vi "PicoReadPicoStreamingBuffers.vi"(1 "enabled array":i16[](array[numeric]), 2 "Buffer and Transfer Settings":T2 {"Down-Sample Mode" items=["None", "Aggregate", "Decimate", "Average"]; "Down Sample Ratio" step=1; "Samples" format="%_6p"}, 3 "Variant":string, 5 "Pointer array":u64[][](array[numeric]), 7 "Offset Index":u32, 9 "Number of Samples":u32, 11 "error in (no error)":errorcluster) -> (6 "Buffers (Max or non-aggregated)":T1, 8 "Buffers (Min)":T1, 15 "error out":errorcluster)   [LabVIEW 2009]
doc: "Read data from Picodata buffers for streaming examples"
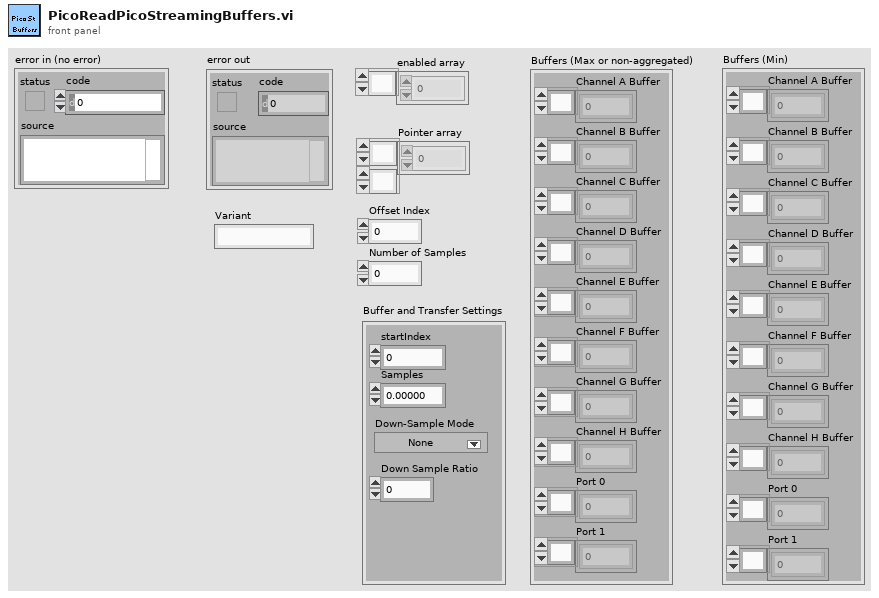
[diagram p1: front panel]
types:
  T1 = cluster{"Channel A Buffer":i16[], "Channel B Buffer":i16[], "Channel C Buffer":i16[], "Channel D Buffer":i16[], "Channel E Buffer":i16[], "Channel F Buffer":i16[], "Channel G Buffer":i16[], "Channel H Buffer":i16[], "Port 0":i16[], "Port 1":i16[]}
  T2 = cluster{"startIndex":u64, "Samples":u64, "Down Sample Ratio":u64, "Down-Sample Mode":u32}
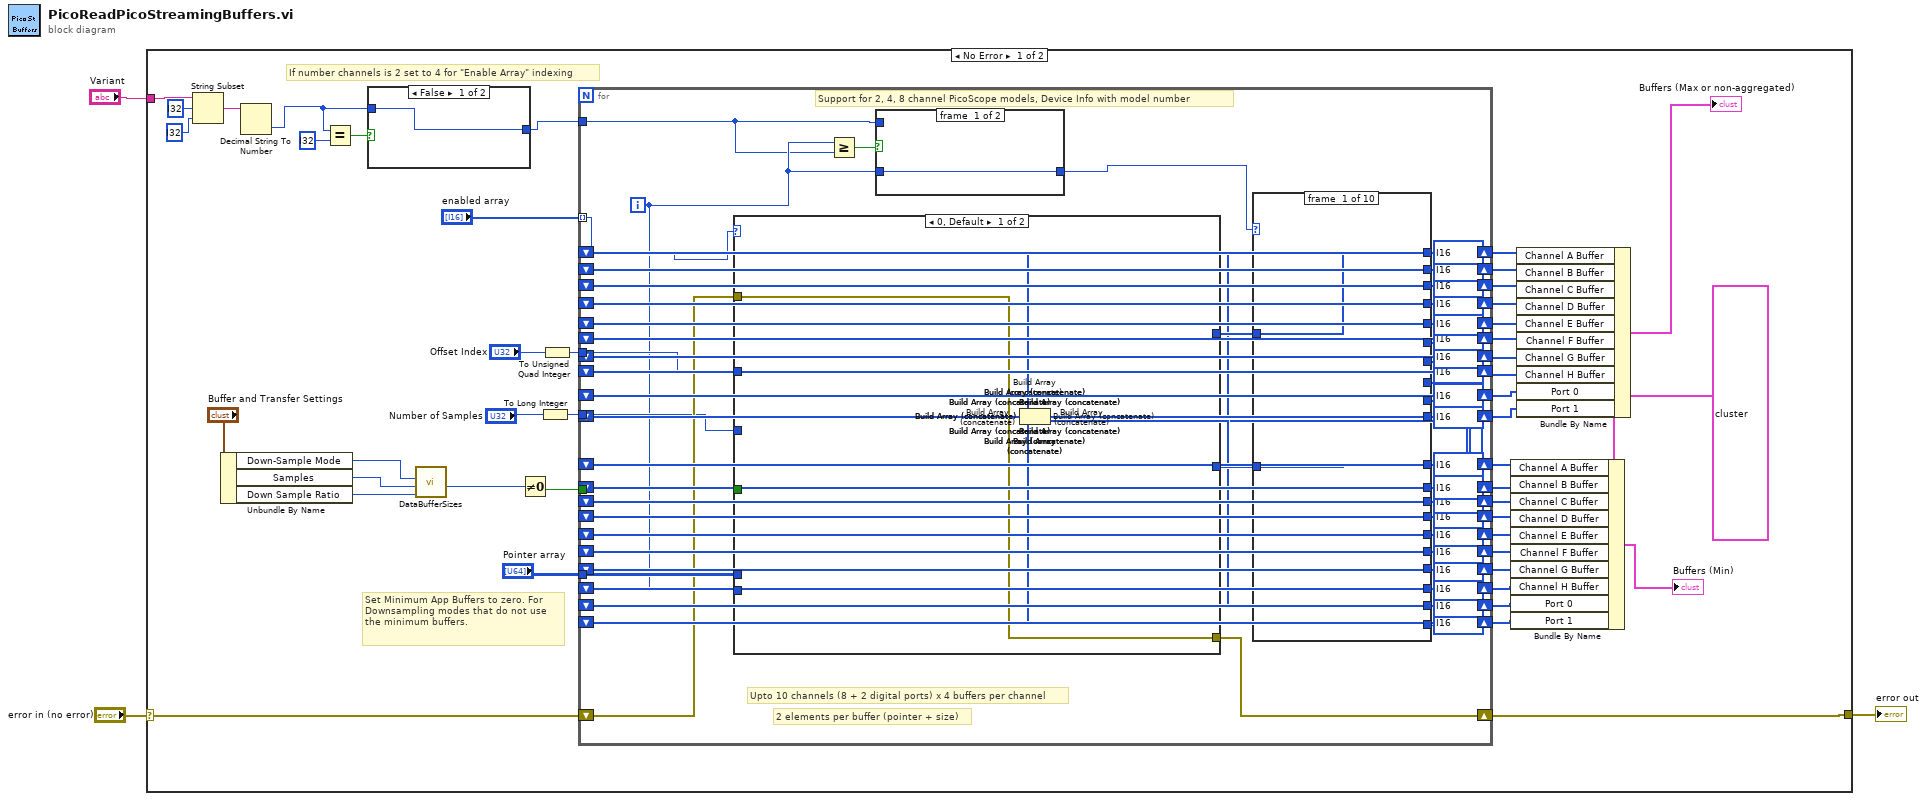
[diagram p0: block diagram]
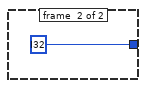
[diagram p2: hidden frame]
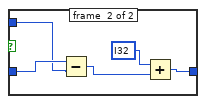
[diagram p3: hidden frame]
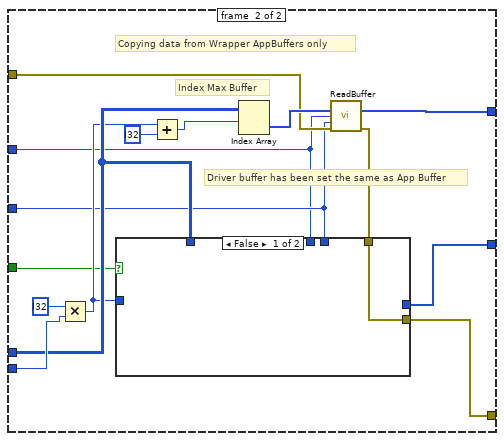
[diagram p13: hidden frame]
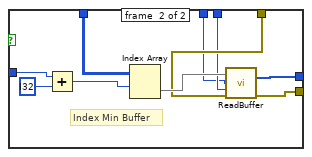
[diagram p14: hidden frame]
diagram:
  n1 = case shown="No Error" "error in (no error)" {
    selector: "error in (no error)" -> [w64 w197]
    tunnel: [w66 w197] -> w2
    tunnel: "Variant" -> [w28 _]
    frame #0 {
      w41 = T1 ? ("Buffers (Max or non-aggregated)")
      # "If number channels is 2 set to 4 for \"Enable Array\" indexing"
      # "Set Minimum App Buffers to zero. For Downsampling modes that do not use the minimum buffers."
      n2 = String Subset(string=w28, offset (0)=i32 ?, length (rest)=i32 ? ("length (rest)")) -> (substring=w25:string)
      n3 = Unbundle By Name("Buffer and Transfer Settings") -> ("Down-Sample Mode"=w51:u32, "Samples"=w50:u64, "Down Sample Ratio"=w52:u64)
      n4 = Decimal String To Number(string=w25) -> (number=w24:i32)  [unwired: 2 in, 1 out]
      n5 = Equal?(x=w24, y=i32 ? ("Number of channels")) -> (x = y?=w31:bool)
      n6 = case shown="False" w31 {
        tunnel: [w69 i32 ? ("Number of channels")] -> w30
        tunnel: w24 -> [w69 _]
        frame #0 {
        }
        frame #1 {
        }
      }
      n7 = call "DataBufferSizes.vi"("Down Sample Ratio"=w52, "Number of Samples"=w50, "Down-Sample Mode"=w51) -> ("min Buffer Size"=w48:i32)  [unwired: 7 in, 1 out]
      n8 = Not Equal To 0?(x=w48) -> (x != 0?=w49:bool)
      n9 = To Long Integer(number="Number of Samples") -> (32bit integer=w43:i32)
      n10 = To Unsigned Quad Integer(1:"Offset Index") -> (0:w46:u64)
      n11 = for {
        tunnel: "enabled array" -> [w142] mode=indexing
        tunnel: "Pointer array" -> [w143]
        shift-right: [w141] -> w66
        shift-left: w64 -> [w140]
        tunnel: w43 -> [w126]
        tunnel: w49 -> [w125]
        tunnel: w46 -> [w123]
        tunnel: w30 -> [w111]
        shift-right: [w109] -> w63
        shift-left: i16[] ? ("Output Array") -> [w110]
        shift-right: [w107] -> w62
        shift-left: i16[] ? ("Output Array") -> [w108]
        shift-right: [w105] -> w61
        shift-left: i16[] ? ("Output Array") -> [w106]
        shift-right: [w103] -> w60
        shift-left: i16[] ? ("Output Array") -> [w104]
        shift-right: [w101] -> w59
        shift-left: i16[] ? ("Output Array") -> [w102]
        shift-right: [w99] -> w58
        shift-left: i16[] ? ("Output Array") -> [w100]
        shift-right: [w97] -> w47
        shift-left: i16[] ? ("Output Array") -> [w98]
        shift-right: [w95] -> w57
        shift-left: i16[] ? ("Output Array") -> [w96]
        shift-right: [w93] -> w56
        shift-left: i16[] ? ("Output Array") -> [w94]
        shift-right: [w91] -> w55
        shift-left: i16[] ? ("Output Array") -> [w92]
        shift-right: [w89] -> w54
        shift-left: i16[] ? ("Output Array") -> [w90]
        shift-right: [w87] -> w53
        shift-left: i16[] ? ("Output Array") -> [w88]
        shift-right: [w85] -> w38
        shift-left: i16[] ? ("Output Array") -> [w86]
        shift-right: [w83] -> w37
        shift-left: i16[] ? ("Output Array") -> [w84]
        shift-right: [w81] -> w39
        shift-left: i16[] ? ("Output Array") -> [w82]
        shift-right: [w79] -> w36
        shift-left: i16[] ? ("Output Array") -> [w80]
        shift-right: [w77] -> w35
        shift-left: i16[] ? ("Output Array") -> [w78]
        shift-right: [w75] -> w34
        shift-left: i16[] ? ("Output Array") -> [w76]
        shift-right: [w73] -> w33
        shift-left: i16[] ? ("Output Array") -> [w74]
        shift-right: [w71] -> w32
        shift-left: i16[] ? ("Output Array") -> [w72]
        i -> [w113]
        # "Support for 2, 4, 8 channel PicoScope models, Device Info with model number"
        # "2 elements per buffer (pointer + size)"
        # "Upto 10 channels (8 + 2 digital ports) x 4 buffers per channel"
        n12 = case shown="0, Default" w142 {
          tunnel: w143 -> [_ w183]
          tunnel: w113 -> [_ w184]
          tunnel: [_ w178] -> w139
          tunnel: [_ w177] -> w138
          tunnel: w140 -> [w170 w176]
          tunnel: [w170 w174] -> w141
          tunnel: w126 -> [_ w172]
          tunnel: w125 -> [_ w173]
          tunnel: w123 -> [_ w171]
          frame #0 {
          }
          frame #1 {
            # "Driver buffer has been set the same as App Buffer"
            # "Copying data from Wrapper AppBuffers only"
            # "Index Max Buffer"
            n13 = Multiply(x=i32 ?, y=w184) -> (x*y=w180:i32)
            n14 = Add(x=w180, y=i32 ?) -> (x+y=w182:i32)
            n15 = Index Array(array=w183, index (row)=w182) -> (element=w179:u64[])  [unwired: 1 in]
            n16 = call "ReadBuffer.vi"("Pointer and BufferSize"=w179, "Offset"=w171, "Buffer size"=w172, "error in (no error)"=w176) -> ("Output Array"=w178:i16[], "error out"=w175:errorcluster)  [unwired: 10 in]
            n17 = case shown="False" w173 {
              tunnel: w183 -> [_ w196]
              tunnel: w180 -> [_ w193]
              tunnel: [_ w191] -> w177
              tunnel: w175 -> [w186 w190]
              tunnel: [w186 w189] -> w174
              tunnel: w172 -> [_ w188]
              tunnel: w171 -> [_ w187]
              frame #0 {
              }
              frame #1 {
                # "Index Min Buffer"
                n18 = Add(x=w193, y=i32 ?) -> (x+y=w194:i32)
                n19 = Index Array(array=w196, index (row)=w194) -> (element=w192:u64[])  [unwired: 1 in]
                n20 = call "ReadBuffer.vi"("Pointer and BufferSize"=w192, "Offset"=w187, "Buffer size"=w188, "error in (no error)"=w190) -> ("Output Array"=w191:i16[], "error out"=w189:errorcluster)  [unwired: 10 in]
              }
            }
          }
        }
        n21 = Greater Or Equal?(x=w113, y=w111) -> (x >= y?=w114:bool)
        n22 = case shown="True" w114 {
          tunnel: w113 -> [w144 w146]
          tunnel: [w144 w148] -> w112
          tunnel: w111 -> [_ w145]
          frame #0 {
          }
          frame #1 {
            n23 = Subtract(x=w146, y=w145) -> (x-y=w147:i32)
            n24 = Add(x=i32 ?, y=w147) -> (x+y=w148:i32)
          }
        }
        n25 = case shown="129" w112 {
          tunnel: w139 -> [w151 w153 w155 w157 w159 w161 w163 w165 w167 w168]
          tunnel: [w151 _ _ _ _ _ _ _ _ _] -> w124
          tunnel: [_ w153 _ _ _ _ _ _ _ _] -> w131
          tunnel: [_ _ w155 _ _ _ _ _ _ _] -> w130
          tunnel: [_ _ _ w157 _ _ _ _ _ _] -> w129
          tunnel: [_ _ _ _ w159 _ _ _ _ _] -> w128
          tunnel: [_ _ _ _ _ w161 _ _ _ _] -> w127
          tunnel: w138 -> [w150 w152 w154 w156 w158 w160 w162 w164 w166 w169]
          tunnel: [w150 _ _ _ _ _ _ _ _ _] -> w137
          tunnel: [_ w152 _ _ _ _ _ _ _ _] -> w136
          tunnel: [_ _ w154 _ _ _ _ _ _ _] -> w135
          tunnel: [_ _ _ w156 _ _ _ _ _ _] -> w134
          tunnel: [_ _ _ _ w158 _ _ _ _ _] -> w133
          tunnel: [_ _ _ _ _ w160 _ _ _ _] -> w132
          tunnel: [_ _ _ _ _ _ w163 _ _ _] -> w122
          tunnel: [_ _ _ _ _ _ _ w165 _ _] -> w121
          tunnel: [_ _ _ _ _ _ w162 _ _ _] -> w120
          tunnel: [_ _ _ _ _ _ _ w164 _ _] -> w119
          tunnel: [_ _ _ _ _ _ _ _ w167 _] -> w118
          tunnel: [_ _ _ _ _ _ _ _ w166 _] -> w117
          tunnel: [_ _ _ _ _ _ _ _ _ w169] -> w116
          tunnel: [_ _ _ _ _ _ _ _ _ w168] -> w115
          frame #0 {
          }
          frame #1 {
          }
          frame #2 {
          }
          frame #3 {
          }
          frame #4 {
          }
          frame #5 {
          }
          frame #6 {
          }
          frame #7 {
          }
          frame #8 {
          }
          frame #9 {
          }
        }
        n26 = Build Array (concatenate)(w72, w115) -> (w71:i16[])
        n27 = Build Array (concatenate)(w74, w116) -> (w73:i16[])
        n28 = Build Array (concatenate)(w76, w117) -> (w75:i16[])
        n29 = Build Array (concatenate)(w78, w118) -> (w77:i16[])
        n30 = Build Array (concatenate)(w80, w119) -> (w79:i16[])
        n31 = Build Array (concatenate)(w82, w120) -> (w81:i16[])
        n32 = Build Array (concatenate)(w84, w121) -> (w83:i16[])
        n33 = Build Array (concatenate)(w86, w122) -> (w85:i16[])
        n34 = Build Array (concatenate)(w88, w127) -> (w87:i16[])
        n35 = Build Array (concatenate)(w90, w128) -> (w89:i16[])
        n36 = Build Array (concatenate)(w92, w129) -> (w91:i16[])
        n37 = Build Array (concatenate)(w94, w130) -> (w93:i16[])
        n38 = Build Array (concatenate)(w96, w131) -> (w95:i16[])
        n39 = Build Array (concatenate)(w98, w124) -> (w97:i16[])
        n40 = Build Array (concatenate)(w100, w132) -> (w99:i16[])
        n41 = Build Array (concatenate)(w102, w133) -> (w101:i16[])
        n42 = Build Array (concatenate)(w104, w134) -> (w103:i16[])
        n43 = Build Array (concatenate)(w106, w135) -> (w105:i16[])
        n44 = Build Array (concatenate)(w108, w136) -> (w107:i16[])
        n45 = Build Array (concatenate)(w110, w137) -> (w109:i16[])
      }
      n46 = Bundle By Name(cluster=w41, "Channel A Buffer"=w63, "Channel B Buffer"=w62, "Channel C Buffer"=w61, "Channel D Buffer"=w60, "Channel E Buffer"=w59, "Channel F Buffer"=w58, "Channel G Buffer"=w39, "Channel H Buffer"=w36, "Port 0"=w34, "Port 1"=w33) -> (→"Buffers (Min)":T1)
      n47 = Bundle By Name(cluster=w41, "Channel A Buffer"=w47, "Channel B Buffer"=w57, "Channel C Buffer"=w56, "Channel D Buffer"=w55, "Channel E Buffer"=w54, "Channel F Buffer"=w53, "Channel G Buffer"=w38, "Channel H Buffer"=w37, "Port 0"=w35, "Port 1"=w32) -> (→"Buffers (Max or non-aggregated)":T1)
    }
    frame #1 {
    }
  }
  "error out" <- w2
